vi "Delete Oneof Template Files.vi"(8 "error in (no error)":errorcluster, 11 "Library in":refnum<vi>) -> (0 "error out":errorcluster, 3 "Library out":refnum<vi>)   [LabVIEW 2019, in "gRPC Template Creation Utility.lvlib"]
uses:
  gRPC Template Creation Utility.lvlib
  OneOf Constants/OneOfConstantsEnum.ctl
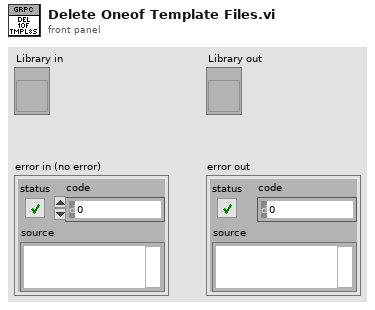
[diagram p1: front panel]
types:
  T1 = typedef "gRPC Template Creation Utility.lvlib/OneOfConstantsEnum.ctl" = enum16{"FlatToRichVIPrefix", "RichToFlatVIPrefix", "FlatTypeDefSuffix"}
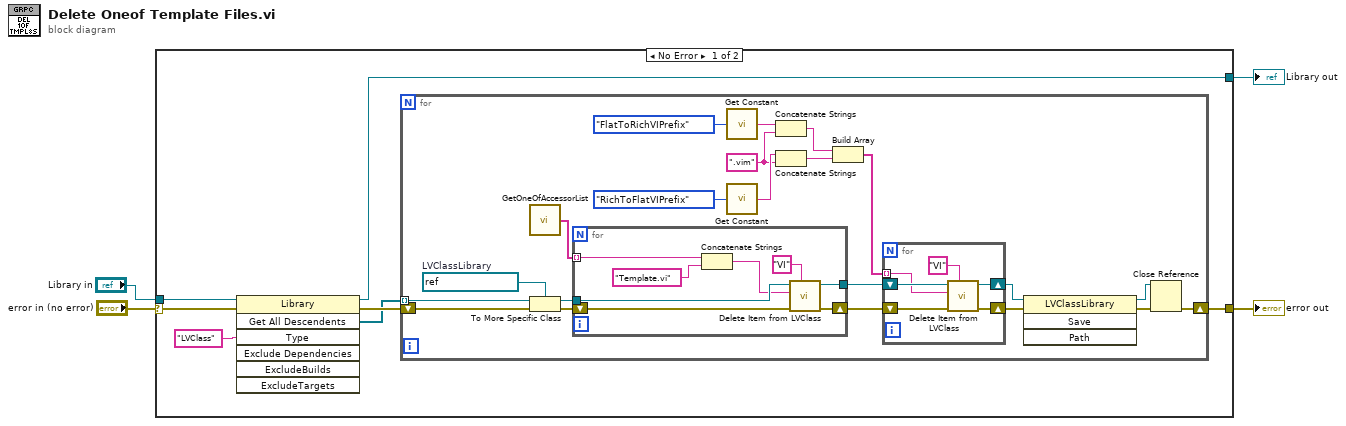
[diagram p0: block diagram]
diagram:
  n1 = case shown="No Error" "error in (no error)" {
    selector: "error in (no error)" -> [w6 w48]
    tunnel: "Library in" -> [w8 w47]
    tunnel: [w7 w47] -> w3
    tunnel: [w5 w48] -> w1
    frame No Error {
      n2 = invoke class="Library" method="Get All Descendents"(reference=w8, error in=w6, "Type"="LVClass") -> (reference out=w7:refnum<vi>, error out=w11:errorcluster, "All Descendents"=w10:refnum<vi>[])  [unwired: 4 in, 4 out]
      n3 = for {
        tunnel: w10 -> [w31] mode=indexing
        shift-right: [w26] -> w5
        shift-left: w11 -> [w28]
        w16 = ".vim" ("string")
        w30 = refnum<vi> refnum  # LVClassLibrary
        n4 = call "GetOneOfAccessorList.vi"() -> ("Array"=w32:string[])
        n5 = To More Specific Class(target class=w30, reference=w31, error in=w28) -> (specific class reference=w29:refnum<vi>, error out=w27:errorcluster)
        n6 = for {
          tunnel: w32 -> [w46] mode=indexing
          tunnel: w29 -> [w44]
          shift-right: [w40] -> w23
          shift-left: w27 -> [w41]
          tunnel: [w39] -> w25
          n7 = Concatenate Strings(w46, "Template.vi" ("string")) -> (w43:string)
          n8 = call "Delete Item from LVClass.vi"("Item Type"="VI", "error in (no error)"=w41, "Item name"=w43, "LVClassLibrary in"=w44) -> ("error out"=w40:errorcluster, "LVClassLibrary out"=w39:refnum<vi>)  [unwired: 5 in, 1 out]
        }
        n9 = call "Get Constant.vi"("Selection"=OneOfConstantsEnum."FlatToRichVIPrefix") -> ("String"=w21:string)
        n10 = call "Get Constant.vi"("Selection"=OneOfConstantsEnum."RichToFlatVIPrefix") -> ("String"=w19:string)
        n11 = Concatenate Strings(w21, w16) -> (w20:string)
        n12 = Concatenate Strings(w19, w16) -> (w17:string)
        n13 = Build Array(w20, w17) -> (w15:string[])
        n14 = for {
          shift-right: [w37] -> w24
          shift-left: w25 -> [w38]
          shift-right: [w35] -> w13
          shift-left: w23 -> [w36]
          tunnel: w15 -> [w34] mode=indexing
          n15 = call "Delete Item from LVClass.vi"("Item Type"="VI", "error in (no error)"=w36, "Item name"=w34, "LVClassLibrary in"=w38) -> ("error out"=w35:errorcluster, "LVClassLibrary out"=w37:refnum<vi>)  [unwired: 5 in, 1 out]
        }
        n16 = invoke class="LVClassLibrary" method="Save"(reference=w24, error in=w13) -> (reference out=w14:refnum<vi>, error out=w12:errorcluster)  [unwired: 2 in, 2 out]
        n17 = Close Reference(reference=w14, error in (no error)=w12) -> (error out=w26:errorcluster)
      }
    }
    frame Error {
    }
  }
  "Library out" <- w3
  "error out" <- w1
